vi "Append _Log_Record.vi"(10 "Record String":string, 11 "Log File":path) -> (0 "error out":errorcluster, 3 "Resolved Log Path":path)   [LabVIEW 2026]
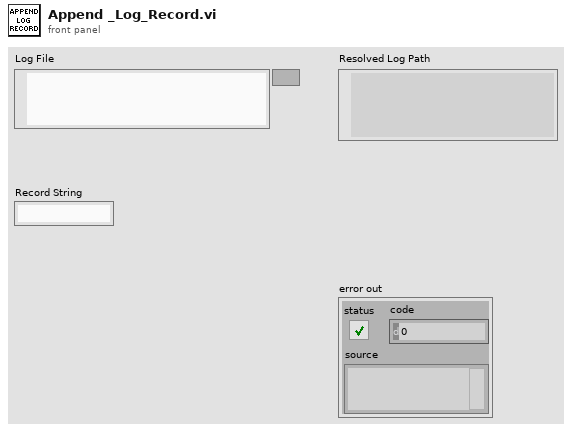
[diagram p1: front panel]
types:
  T1 = enum16{"open", "replace", "create", "open or create", "replace or create", "replace or create with confirmation"}
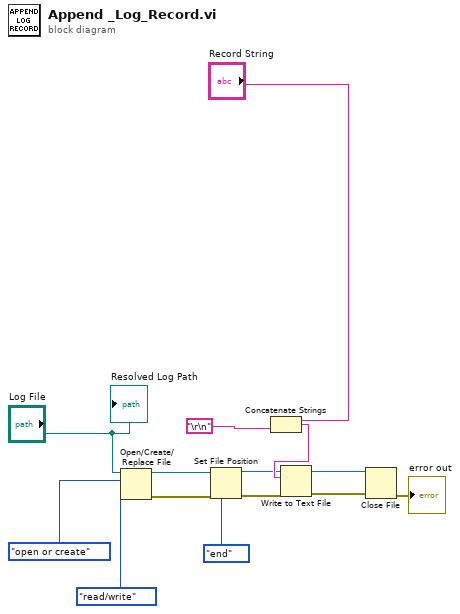
[diagram p0: block diagram]
diagram:
  n1 = Open/Create/Replace File(file path (use dialog)="Log File", operation (0:open)=T1."open or create", access (0:read/write)=enum16{"read/write", "read-only", "write-only"}."read/write") -> (refnum out=w1:refnum<file>, error out=w6:errorcluster)  [unwired: 3 in, 1 out]
  n2 = Set File Position(refnum=w1, from (0:start)=enum16{"start", "end", "current"}."end", error in=w6) -> (refnum out=w2:refnum<file>, error out=w7:errorcluster)  [unwired: 1 in]
  n3 = Concatenate Strings("Record String", "\r\n") -> (w14:string)
  n4 = Write to Text File(file (use dialog)=w2, text=w14, error in=w7) -> (refnum out=w5:refnum<file>, error out=w8:errorcluster)  [unwired: 1 in, 1 out]
  n5 = Close File(refnum=w5, error in=w8) -> (error out=→"error out":errorcluster)  [unwired: 1 out]
  "Resolved Log Path" <- "Log File"
